vi "Create Digraph String.vi"(10 "node connections":string[][](array[string]), 11 "tables html":string[](array[string])) -> (3 "digraph output":string)   [LabVIEW 2014, in "GraphViz Mapping Visualizer.lvlib"]
uses:
  GraphViz Mapping Visualizer.lvlib
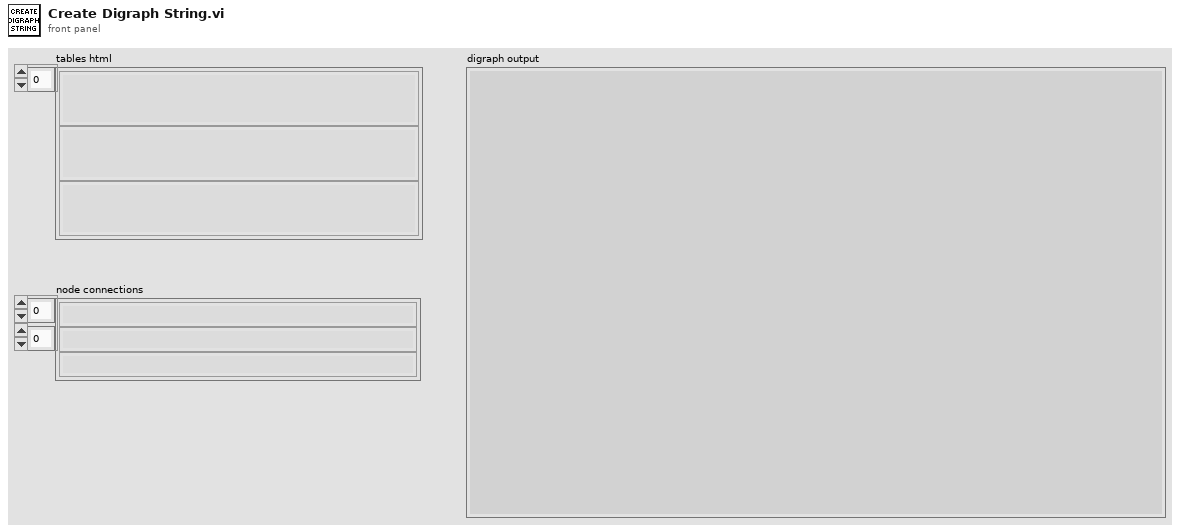
[diagram p1: front panel]
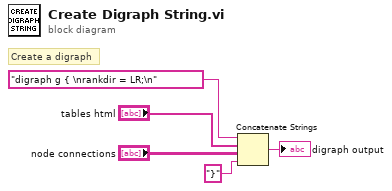
[diagram p0: block diagram]
diagram:
  # "Create a digraph"
  n1 = Concatenate Strings("digraph g { \nrankdir = LR;\n", "tables html", "node connections", "}") -> (→"digraph output":string)
